vi "consoleUi.vi"(8 "error in (no error)":errorcluster, 11 "Handler.UserEvent.Console in":refnum<class "Handler.UserEvent.Console.lvclass">) -> (0 "error out":errorcluster, 2 "Display User Event Logs":string, 3 "Handler.UserEvent.Console out":refnum<class "Handler.UserEvent.Console.lvclass">)   [LabVIEW 2017, in "Error Log.lvlib" / "Handler.UserEvent.Console.lvclass"]
uses:
  Handler.UserEvent.Console.lvclass
  \\192.168.1.40\Neosoft/Partage/Dossiers Personnels/BRO/DevTools_BR/wc/ErrorLog/src/Handler.UserEvent/Handler.UserEvent.lvclass
  \\192.168.1.40\Neosoft/Partage/Dossiers Personnels/BRO/DevTools_BR/wc/ErrorLog/src/Handler/Handler.lvclass
  Handler.UserEvent/Handler.UserEvent.lvclass/Handler.UserEvent.ctl
  Handler.UserEvent.Console.lvclass/Handler.UserEvent.Console.ctl
  Handler/Handler.lvclass/Handler.ctl
  Record/Record.lvclass/Record.ctl
  Record/Get Level.vi
  Handler.UserEvent/Get New Record.vi
  Get Private Events.vi
  Get Style Color.vi
  Handler/Get Caller VI Ref.vi
  Handler/Get Level.vi
  Record/Record.lvclass
panel:
  out "MsgLevel":string
  in  "Settings":bool
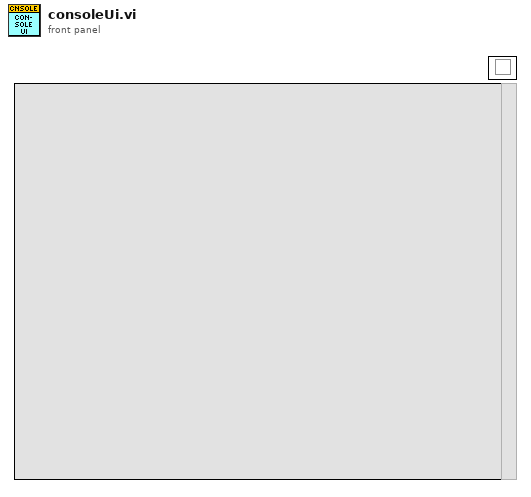
[diagram p1: front panel]
types:
  T1 = enum32{"Invalid", "Standard", "Closed", "Hidden", "Minimized", "Maximized"}
  T2 = typedef "Error Log.lvlib/Handler.UserEvent.Console.lvclass/privateEvents.ctl" = cluster{"Stop":refnum<user-event>, "Show Hide UI":refnum<user-event>, "Clear":refnum<user-event>}
  T3 = enum16{"DEBUG", "INFO", "WARNING", "ERROR", "CRITICAL"}
  T4 = cluster{"Public API:Properties:New Record":refnum<user-event>, "Public API:Properties:Private Events":T2}
  T5 = enum32{"Bad", "Idle", "Run top level", "Running"}
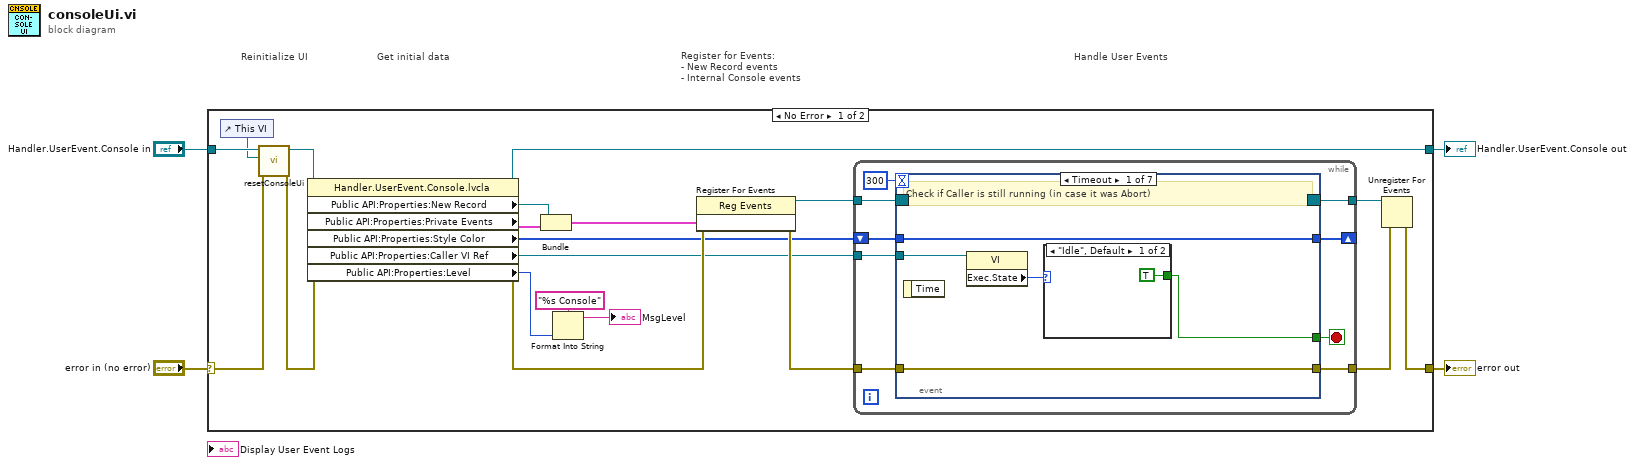
[diagram p0: block diagram]
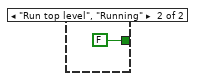
[diagram p2: hidden frame]
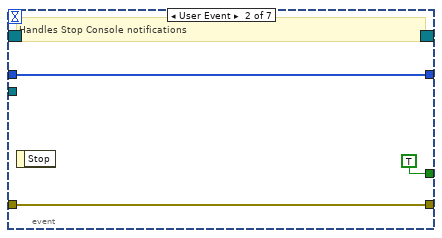
[diagram p3: hidden frame]
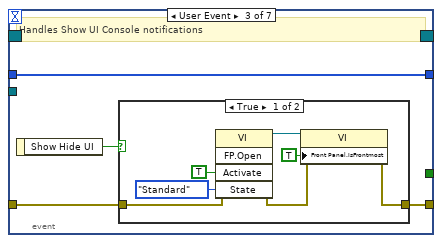
[diagram p4: hidden frame]
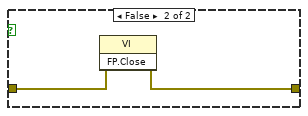
[diagram p5: hidden frame]
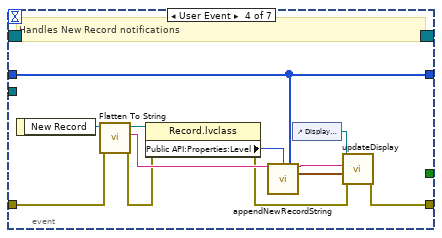
[diagram p6: hidden frame]
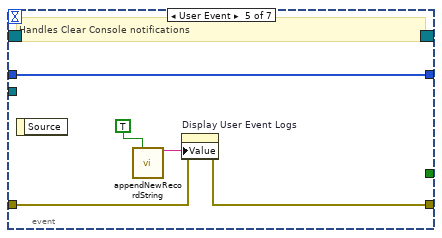
[diagram p7: hidden frame]
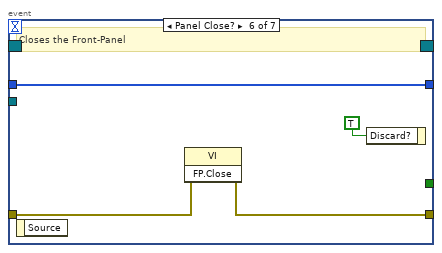
[diagram p8: hidden frame]
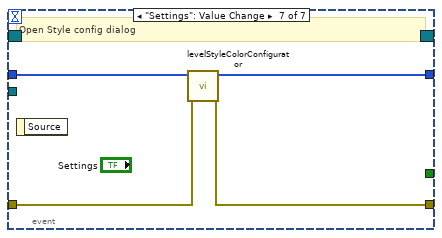
[diagram p9: hidden frame]
diagram:
  # "Handle User Events"
  # "Get initial data"
  # "Register for Events:\n- New Record events\n- Internal Console events"
  # "Reinitialize UI"
  n1 = case shown="No Error" "error in (no error)" {
    selector: "error in (no error)" -> [w13 w83]
    tunnel: [w18 w83] -> w3
    tunnel: [w16 w82] -> w1
    tunnel: "Handler.UserEvent.Console in" -> [w15 w82]
    frame No Error {
      n2 = control-ref of="This VI"() -> (w11:refnum<vi>)
      n3 = call "resetConsoleUi.vi"("error in (no error)"=w13, "reference"=w11, "Handler.UserEvent.Console in"=w15) -> ("error out"=w12:errorcluster, "Handler.UserEvent.Console out"=w14:refnum<class "Handler.UserEvent.Console.lvclass">)  [unwired: 7 in]
      n4 = property class="Handler.UserEvent.Console.lvcla"(reference=w14, error in=w12) -> (reference out=w16:refnum<class "Handler.UserEvent.Console.lvclass">, error out=w9:errorcluster, "Public API:Properties:New Record"=w24:refnum<user-event>, "Public API:Properties:Private Events"=w23:T2, "Public API:Properties:Style Color"=w8:u32[], "Public API:Properties:Caller VI Ref"=w6:refnum<vi>, "Public API:Properties:Level"=w7:T3)
      n5 = Bundle("Public API:Properties:New Record"=w24, "Public API:Properties:Private Events"=w23) -> (w22:T4)  [unwired: 1 in]
      n6 = Format Into String(format string="%s Console", w7) -> (resulting string=→"MsgLevel":string)  [unwired: 2 in, 1 out]
      n7 = register-events(error in=w9, w22) -> (reference out=w21:refnum<event-registration>, error out=w17:errorcluster)  [unwired: 1 in]
      n8 = while {
        tunnel: w21 -> [w33]
        tunnel: w17 -> [w31]
        tunnel: [w30] -> w19
        tunnel: [w29] -> w20
        shift-right: [w28] -> _
        shift-left: w8 -> [w27]
        tunnel: w6 -> [w26]
        stop <- w32 stop-if-true
        n9 = event shown="[0] Timeout" {
          selector: w33 -> [_ _ _ _ _ _ _]
          dyn-events: [_ _ _ _ _ _ _] -> w29
          timeout: 300 -> [_ _ _ _ _ _ _]
          tunnel: [w34 TRUE _ _ _ _ _] -> w32
          tunnel: w31 -> [w38 w42 w46 w67 w73 w77 w79]
          tunnel: [w38 w42 w45 w59 w72 w76 w78] -> w30
          tunnel: [w37 w41 w44 w60 w69 w74 w81] -> w28
          tunnel: w27 -> [w37 w41 w44 w60 w69 w74 w80]
          tunnel: w26 -> [w36 _ _ _ _ _ _]
          event Timeout {
            # "Check if Caller is still running (in case it was Abort)"
            n10 = event-data() -> ()  [unwired: 1 in, 1 out]
            n11 = property class="VI"(reference=w36) -> ("Exec.State"=w35:T5)  [unwired: 1 in, 2 out]
            n12 = case shown="\"Idle\", Default" w35 {
              tunnel: [TRUE FALSE] -> w34
              frame "Idle", Default {
              }
              frame "Run top level", "Running" {
              }
            }
          }
          event User Event {
            # "Handles Stop Console notifications"
            n13 = event-data() -> ()  [unwired: 1 in, 1 out]
          }
          event User Event {
            # "Handles Show UI Console notifications"
            n14 = event-data() -> ("Show Hide UI"=w47:bool)  [unwired: 1 in]
            n15 = case shown="True" w47 {
              tunnel: w46 -> [w52 w56]
              tunnel: [w48 w55] -> w45
              frame True {
                n16 = invoke class="VI" method="FP.Open"(error in=w52, "Activate"=TRUE ("Activate?"), "State"=T1."Standard") -> (reference out=w51:refnum<vi>, error out=w49:errorcluster)  [unwired: 2 in, 3 out]
                n17 = property class="VI"(reference=w51, error in=w49, "Front Panel.IsFrontmost"=TRUE ("Front Panel Window:Is Frontmost")) -> (error out=w48:errorcluster)  [unwired: 1 out]
              }
              frame False {
                n18 = invoke class="VI" method="FP.Close"(error in=w56) -> (error out=w55:errorcluster)  [unwired: 2 in, 2 out]
              }
            }
          }
          event User Event {
            # "Handles New Record notifications"
            n19 = event-data() -> ("New Record"=w68:refnum<class "Record.lvclass">)  [unwired: 1 in]
            n20 = call "Flatten To String.vi"("error in (no error)"=w67, "Record in"=w68) -> ("error out"=w58:errorcluster, "String"=w66:string, "Record out"=w65:refnum<class "Record.lvclass">)  [unwired: 7 in]
            n21 = property class="Record.lvclass"(reference=w65, error in=w58) -> (error out=w57:errorcluster, "Public API:Properties:Level"=w64:T3)  [unwired: 1 out]
            n22 = call "appendNewRecordString.vi"("New Record String"=w66, "Level"=w64, "Style Color"=w60) -> ("Log Display Updated"=w62:string, "Colors"=w63:cluster{"length":u32, "color":u32}[])  [unwired: 11 in]
            n23 = control-ref of="Display User Event Logs"() -> (w61:refnum<vi>)
            n24 = call "updateDisplay.vi"("error in (no error)"=w57, "Display Colors"=w63, "Log Display Updated"=w62, "reference"=w61) -> ("error out"=w59:errorcluster)  [unwired: 7 in]
          }
          event User Event {
            # "Handles Clear Console notifications"
            n25 = event-data() -> ()  [unwired: 1 in, 1 out]
            n26 = call "appendNewRecordString.vi"("clear"=TRUE) -> ("Log Display Updated"=w70:string)  [unwired: 13 in, 1 out]
            n27 = property on="Display User Event Logs" class="Str"(error in=w73, "Value"=w70) -> (error out=w72:errorcluster)  [unwired: 1 in, 1 out]
          }
          event Panel Close? {
            # "Closes the Front-Panel"
            n28 = event-data() -> ()  [unwired: 1 in, 1 out]
            n29 = invoke class="VI" method="FP.Close"(error in=w77) -> (error out=w76:errorcluster)  [unwired: 2 in, 2 out]
            n30 = event-data("Discard?"=TRUE) -> ()  [unwired: 1 in, 1 out]
          }
          event "Settings": Value Change {
            # "Open Style config dialog"
            n31 = event-data() -> ()  [unwired: 1 in, 1 out]
            n32 = call "levelStyleColorConfigurator.vi"("error in (no error)"=w79, "Colors in"=w80) -> ("error out"=w78:errorcluster, "Colors out"=w81:u32[])  [unwired: 8 in]
          }
        }
      }
      n33 = Unregister For Events(event registration refnum=w20, error in=w19) -> (error out=w18:errorcluster)
    }
    frame Error {
    }
  }
  "error out" <- w3
  "Handler.UserEvent.Console out" <- w1
